vi "Define Test Suite (Default).vi"(4 "timeout":i32=2000, 5 "register caller level (0)":i32, 6 "Verbose (F)":bool, 7 "Test Report (optional)":refnum<class "Test Report.lvclass">, 8 "error in (no error)":errorcluster, 10 "Interactive":bool, 11 "Label (VI Title)":string) -> (0 "error out":errorcluster, 2 "Properties.Suite":refnum<class "Properties.Suite.lvclass">, 3 "Test Suite":refnum<class "Test Suite.lvclass">)   [LabVIEW 2020, in "Caraya.lvlib" / "Test Suite.lvclass"]
doc: "Registers the calling VI as a test suite. If Interactive is True, the interactive user interface is opened when the test suite is executed. If the Report Path is set, a report file will be generated with the test results.\n\n--\nCopyright © 2015 JKI All rights reserved.\n\nAuthor: Tomi Maila <tomi.maila@jki.net>\n\nThis library is provided \"AS IS\" ,WITHOUT WARRANTIES OR\nCONDITIONS OF ANY KIND, either express or implied.\n\nJKI -- jki.net"
uses:
  Test Suite.lvclass
  Test Report/Test Report.lvclass
  Properties.Suite/Properties.Suite.lvclass
  C:/projects/caraya/src/classes/Properties/Properties.lvclass
  Test Assert Factory/Test Assert Factory.lvclass
  Test Suite.lvclass/Test Suite.ctl
  Properties.Suite/Properties.Suite.lvclass/Properties.Suite.ctl
  Caraya.lvlib
  Assert Factory Manager/Assert Factory Manager.lvclass
  Basic Test Manager/Basic Test Manager.lvclass
  Properties/Properties.lvclass
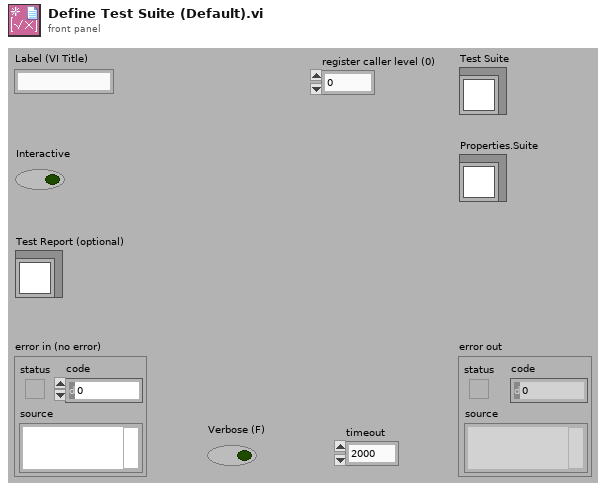
[diagram p1: front panel]
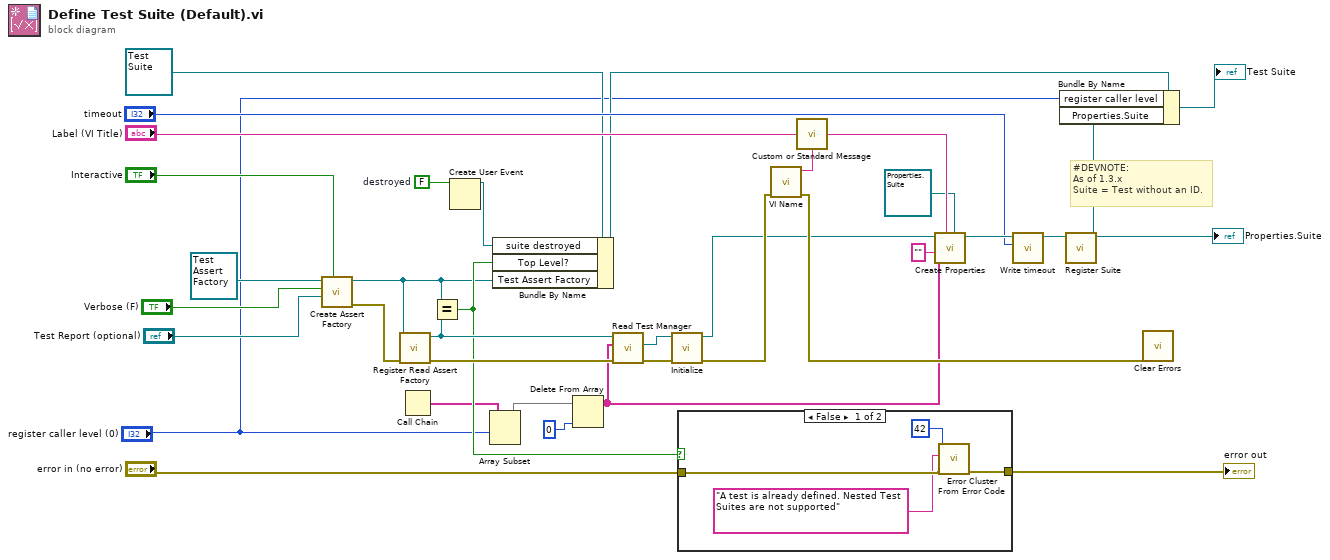
[diagram p0: block diagram]
diagram:
  w17 = FALSE  # destroyed
  # "#DEVNOTE:\nAs of 1.3.x\nSuite = Test without an ID."
  n1 = call "Create Assert Factory.vi"("Interactive"="Interactive", "Test Report"="Test Report (optional)", "Verbose (F)"="Verbose (F)", "Test Assert Factory in"=refnum<class "Test Assert Factory.lvclass"> refnum ("Caraya.lvlib:Test Assert Factory.lvclass")) -> ("error out"=w20:errorcluster, "Test Assert Factory out"=w21:refnum<class "Test Assert Factory.lvclass">)  [unwired: 6 in]
  n2 = call "Register Read Assert Factory.vi"("error in (no error)"=w20, "Test Assert Factory"=w21) -> ("error out"=w34:errorcluster, "Test Assert Factory"=w28:refnum<class "Test Assert Factory.lvclass">)  [unwired: 8 in]
  n3 = Call Chain() -> (call chain=w3:string[])
  n4 = Equal?(x=w21, y=w28) -> (x = y?=w25:bool)
  n5 = Create User Event(user event datatype=w17) -> (user event=w16:refnum<user-event>)  [unwired: 1 in, 1 out]
  n6 = Array Subset(array=w3, index="register caller level (0)") -> (w2:string[])  [unwired: 1 in]
  n7 = Bundle By Name(cluster=refnum<class "Test Suite.lvclass"> refnum ("Test Suite"), "suite destroyed"=w16, "Top Level?"=w25, "Test Assert Factory"=w21) -> (w5:refnum<class "Test Suite.lvclass">)
  n8 = Delete From Array(array=w2, index=0) -> (array with subset deleted=w11:string[])  [unwired: 1 in, 1 out]
  n9 = call-dynamic "Read Test Manager.vi"("error in (no error)"=w34, "VI Call Chain"=w11, "Assert Factory in"=w28) -> ("error out"=w32:errorcluster, "Basic Test Manager"=w24:refnum<class "Basic Test Manager.lvclass">)  [unwired: 6 in, 1 out]
  n10 = call "Initialize.vi"("error in (no error)"=w32, "Test Manager in"=w24) -> ("error out"=w31:errorcluster, "Test Manager out"=w15:refnum<class "Basic Test Manager.lvclass">)  [unwired: 8 in]
  n11 = case shown="False" w25 {
    tunnel: [w39 w40] -> w27
    tunnel: "error in (no error)" -> [w38 w40]
    frame False {
      n12 = call <vilib>:"Error Cluster From Error Code.vi"("error in (no error)"=w38, "error message (\"\")"="A test is already defined. Nested Test Suites are not supported" ("error message (\"\")"), "error code (0)"=42) -> ("error out"=w39:errorcluster)  [unwired: 6 in]
    }
    frame True {
    }
  }
  "error out" <- w27
  n13 = call "VI Name.vi"("error in (no error)"=w31) -> ("error out"=w30:errorcluster, "VI Name"=w33:string)  [unwired: 9 in]
  n14 = call "Custom or Standard Message.vi"("Custom Message"="Label (VI Title)", "Standard Message"=w33) -> ("Message"=w14:string)
  n15 = call "Create Properties.vi"("Properties in"=refnum<class "Properties.Suite.lvclass"> refnum ("Caraya.lvlib:Properties.Suite.lvclass"), "label"=w14, "call-chain"=w11, "self-id"="", "Test Manager"=w15) -> ("Properties out"=w10:refnum<class "Properties.Suite.lvclass">)  [unwired: 6 in]
  n16 = call "Write timeout.vi"("timeout"="timeout", "Properties.Suite in"=w10) -> ("Properties.Suite out"=w9:refnum<class "Properties.Suite.lvclass">)  [unwired: 9 in]
  n17 = call "Register Suite.vi"("Properties.Suite in"=w9) -> ("Properties.Suite out"=w6:refnum<class "Properties.Suite.lvclass">)  [unwired: 10 in]
  "Properties.Suite" <- w6
  n18 = Bundle By Name(cluster=w5, "register caller level"="register caller level (0)", "Properties.Suite"=w6) -> (→"Test Suite":refnum<class "Test Suite.lvclass">)
  n19 = call <vilib>:"Clear Errors.vi"("error in (no error)"=w30) -> ()  [unwired: 5 in, 2 out]
